vi "TypeSpeficifer.vi"(8 "error in (no error)":errorcluster, 11 "Channel":refnum<class "Channel.lvclass">) -> (0 "error out":errorcluster, 3 "Type_Channel":refnum<class "Type_Channel.lvclass">)   [LabVIEW 2021, in "Template-ChannelsChild.lvlib"]
uses:
  Template-ChannelsChild.lvlib
  Type_Channel/Type_Channel.lvclass
  Dependencies/Channel.lvlibp/Channel/Channel_class/Channel.lvclass
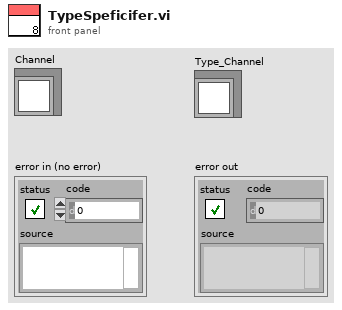
[diagram p1: front panel]
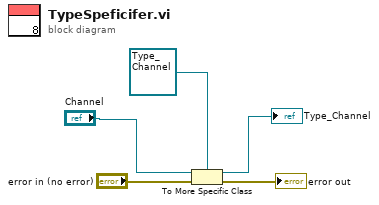
[diagram p0: block diagram]
diagram:
  n1 = To More Specific Class(target class=refnum<class "Type_Channel.lvclass"> refnum ("Type_Channel"), reference="Channel", error in="error in (no error)") -> (specific class reference=→"Type_Channel":refnum<class "Type_Channel.lvclass">, error out=→"error out":errorcluster)
